vi "Test Comm CAN.vi"() -> ()   [LabVIEW 2021]
uses:
  <vilib>/CIF Foundation/CIF Channels Core/ChannelCommon/typedef/Direction.ctl
  CIF_CIPC_CAN.lvclass
  <vilib>/CIF Foundation/CIF Channels Core/ChannelCommon/typedef/FIFO Config.ctl
  <vilib>/CIF Foundation/CIF Channels Core/ChannelCommon/typedef/TimeStamps.ctl
  <vilib>/CIF Foundation/CIF Channels Core/ChannelCommon/typedef/New FIFO Instance Configuration.ctl
  <vilib>/CIF Foundation/CIF Channels Core/ChannelCommon/ChannelCommon.lvlib
panel:
  out "status":string
  out "pass":bool
  out "error out":errorcluster
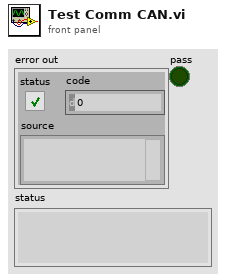
[diagram p1: front panel]
types:
  T1 = typedef "ChannelCommon.lvlib/Direction.ctl" = enum8{"Publisher", "Subscriber"}
  T2 = typedef "ChannelCommon.lvlib/New FIFO Instance Configuration.ctl" = cluster{"Backpressure":bool, "Bytes/Message Override":u32, "Messages/FIFO Override":u32, "Custom Data":u8[]}
  T3 = typedef "ChannelCommon.lvlib/TimeStamps.ctl" = cluster{"ClockID":u8, "T0":i64, "T_Out":i64}
  T4 = typedef "ChannelCommon.lvlib/FIFO Config.ctl" = cluster{"Max Bytes/Msg":u64, "Max Msg/FIFO":u64, "Flags":u64, "Custom Data":u8[]}
  T5 = typedef "ChannelCommon.lvlib/New FIFO Instance Response.ctl" = cluster{"Publisher":string, "Custom Data":u8[]}
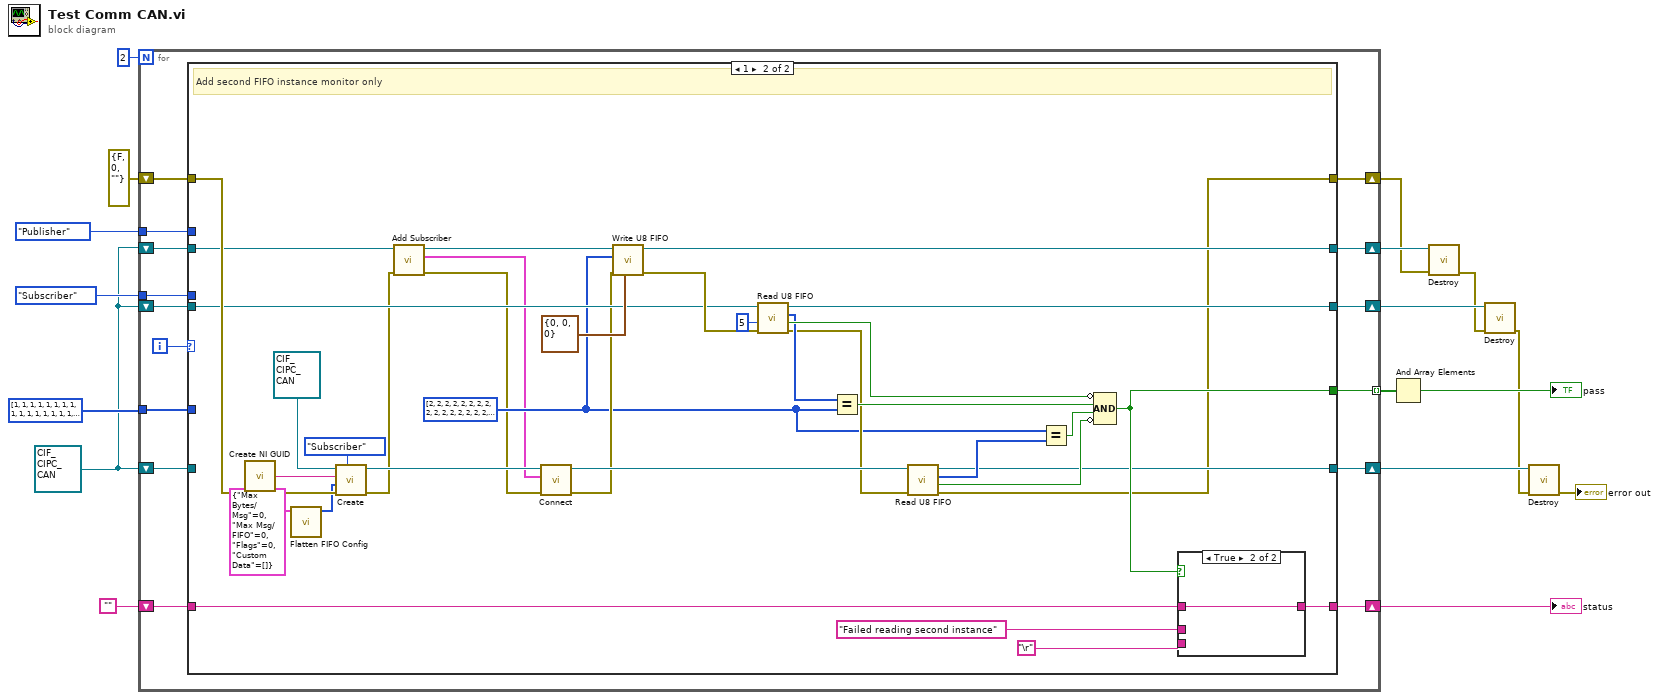
[diagram p0: block diagram]
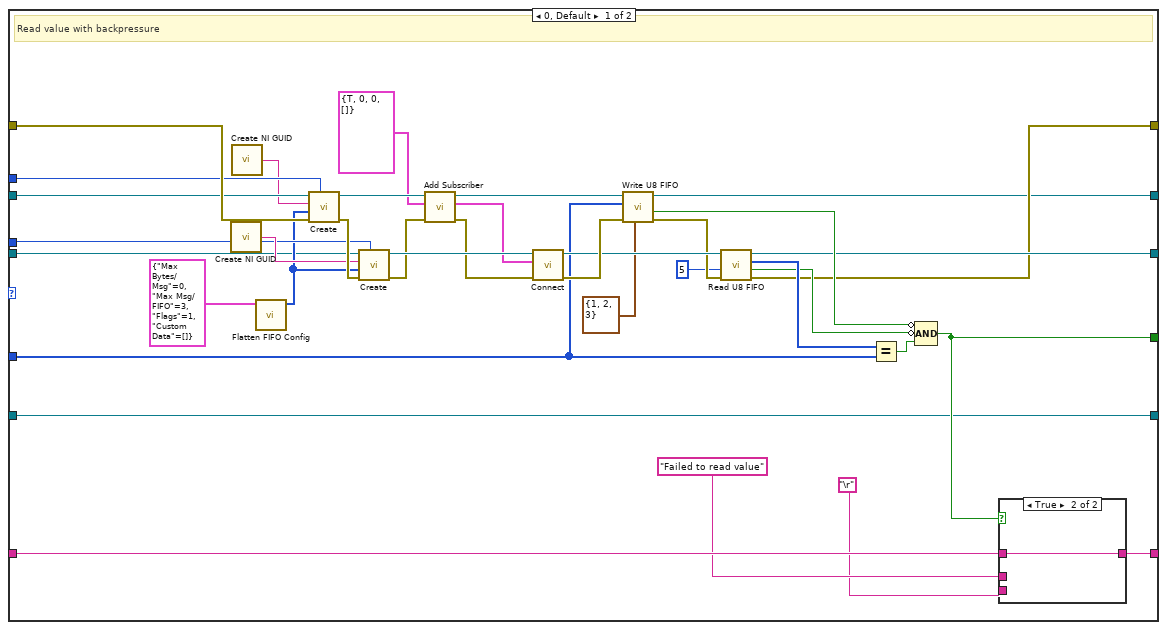
[diagram p2: hidden frame]
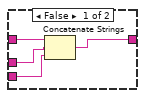
[diagram p3: hidden frame]
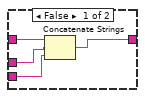
[diagram p4: hidden frame]
diagram:
  w1 = refnum<class "CIF_CIPC_CAN.lvclass"> refnum ("CIF_DAQ_DVR_Multi.lvclass")
  n1 = for {
    N: 2 -> [_]
    tunnel: [w32] -> w17 mode=indexing
    shift-right: [w25] -> w7
    shift-left: errorcluster {"status"=FALSE, "code"=0, "source"=""} ("error out") -> [w31]
    shift-right: [w28] -> w13
    shift-left: "" -> [w29]
    tunnel: Direction."Subscriber" ("Direction") -> [w27]
    tunnel: Direction."Publisher" ("Direction") -> [w26]
    shift-right: [w20] -> w9
    shift-left: w1 -> [w24]
    shift-right: [w19] -> w8
    shift-left: w1 -> [w18]
    tunnel: u8[] [1, 1, 1, 1, 1, 1, 1, 1, 1, 1, 1, 1, 1, 1, 1, 1, 1, 1, 1, 1, 1, 1, 1, 1, 1, 1, 1, 1, 1, 1, 1, 1, 1, 1, 1, 1, 1, 1, 1, 1, 1, 1, 1, 1, 1, 1, 1, 1, 1, 1, 1] ("Data in") -> [w23]
    shift-right: [w21] -> w5
    shift-left: w1 -> [w22]
    i -> [w30]
    n2 = case shown="1" w30 {
      tunnel: [w63 w104] -> w32
      tunnel: w31 -> [w61 w94]
      tunnel: [w42 w80] -> w25
      tunnel: w29 -> [w68 w108]
      tunnel: [w67 w107] -> w28
      tunnel: w27 -> [w59 _]
      tunnel: w26 -> [w58 _]
      tunnel: [w43 w86] -> w20
      tunnel: [w40 w84] -> w19
      tunnel: w18 -> [w48 w78]
      tunnel: w24 -> [w47 w85]
      tunnel: w23 -> [w41 _]
      tunnel: w22 -> [w46 _]
      tunnel: [w46 w87] -> w21
      frame 0, Default {
        # "Read value with backpressure"
        n3 = call <vilib>:"Create NI GUID.vi"() -> ("NI GUID"=w60:string)
        n4 = call <vilib>:"Create NI GUID.vi"() -> ("NI GUID"=w37:string)
        n5 = call <vilib>:"Flatten FIFO Config.vi"("FIFO Config in"=T4 {"Max Bytes/Msg"=0, "Max Msg/FIFO"=3, "Flags"=1, "Custom Data"=[]}) -> ("Flattened FIFO Config"=w55:u8[])  [unwired: 10 in]
        n6 = call-dynamic "Create.vi"("Direction"=w58, "error in (no error)"=w61, "Custom Config Data"=w55, "Name"=w37, "CIFFIFO in"=w48) -> ("error out"=w62:errorcluster, "CIFFIFO out"=w39:refnum<class "CIF_CIPC_CAN.lvclass">)  [unwired: 5 in]
        n7 = call-dynamic "Create.vi"("Direction"=w59, "error in (no error)"=w62, "Custom Config Data"=w55, "Name"=w60, "CIFFIFO in"=w47) -> ("error out"=w34:errorcluster, "CIFFIFO out"=w56:refnum<class "CIF_CIPC_CAN.lvclass">)  [unwired: 5 in]
        n8 = call-dynamic "Add Subscriber.vi"("error in (no error)"=w34, "New FIFO Instance Config"=T2 {"Backpressure"=TRUE, "Bytes/Message Override"=0, "Messages/FIFO Override"=0, "Custom Data"=[]}, "CIF_CIPC_Chn in"=w39) -> ("error out"=w33:errorcluster, "New FIFO Instance"=w36:T5, "CIF_CIPC_Chn out"=w38:refnum<class "CIF_CIPC_CAN.lvclass">)  [unwired: 6 in]
        n9 = call-dynamic "Connect.vi"("error in (no error)"=w33, "Connection"=w36, "CIFTag in"=w56) -> ("error out"=w54:errorcluster, "CIFTag out"=w52:refnum<class "CIF_CIPC_CAN.lvclass">)  [unwired: 7 in]
        n10 = call-dynamic "Write U8 FIFO.vi"("FIFO Timestamps"=T3 {"ClockID"=1, "T0"=2, "T_Out"=3}, "error in (no error)"=w54, "Data in"=w41, "CIFFIFO in"=w38) -> ("error out"=w49:errorcluster, "timed out?"=w53:bool, "CIFFIFO out"=w40:refnum<class "CIF_CIPC_CAN.lvclass">)  [unwired: 4 in, 1 out]
        n11 = call-dynamic "Read U8 FIFO.vi"("error in (no error)"=w49, "Timeout (ms)"=5, "CIFFIFO in"=w52) -> ("error out"=w42:errorcluster, "timed out?"=w50:bool, "Data out"=w51:u8[], "CIFFIFO out"=w43:refnum<class "CIF_CIPC_CAN.lvclass">)  [unwired: 4 in, 1 out]
        n12 = Equal?(x=w51, y=w41) -> (x = y?=w64:bool)
        n13 = Compound Arithmetic op=AND(invert w53, invert w50, w64) -> (w63:bool)
        n14 = case shown="True" w63 {
          tunnel: w68 -> [w72 w73]
          tunnel: [w69 w73] -> w67
          tunnel: "Failed to read value" -> [w71 _]
          tunnel: "\r" -> [w70 _]
          frame False {
            n15 = Concatenate Strings(w72, w71, w70) -> (w69:string)
          }
          frame True {
          }
        }
      }
      frame 1 {
        w79 = u8[] [2, 2, 2, 2, 2, 2, 2, 2, 2, 2, 2, 2, 2, 2, 2, 2, 2, 2, 2, 2, 2, 2, 2, 2, 2, 2, 2, 2, 2, 2, 2, 2, 2, 2, 2, 2, 2, 2, 2, 2, 2, 2, 2, 2, 2, 2, 2, 2, 2, 2, 2] ("Data in")
        # "Add second FIFO instance monitor only"
        n16 = call <vilib>:"Create NI GUID.vi"() -> ("NI GUID"=w96:string)
        n17 = call <vilib>:"Flatten FIFO Config.vi"("FIFO Config in"=T4 {"Max Bytes/Msg"=0, "Max Msg/FIFO"=0, "Flags"=0, "Custom Data"=[]}) -> ("Flattened FIFO Config"=w93:u8[])  [unwired: 10 in]
        n18 = call-dynamic "Create.vi"("Direction"=Direction."Subscriber", "error in (no error)"=w94, "Custom Config Data"=w93, "Name"=w96, "CIFFIFO in"=refnum<class "CIF_CIPC_CAN.lvclass"> refnum ("CIF_DAQ_DVR_Multi.lvclass")) -> ("error out"=w77:errorcluster, "CIFFIFO out"=w95:refnum<class "CIF_CIPC_CAN.lvclass">)  [unwired: 5 in]
        n19 = call-dynamic "Add Subscriber.vi"("error in (no error)"=w77, "CIF_CIPC_Chn in"=w78) -> ("error out"=w76:errorcluster, "New FIFO Instance"=w75:T5, "CIF_CIPC_Chn out"=w74:refnum<class "CIF_CIPC_CAN.lvclass">)  [unwired: 7 in]
        n20 = call-dynamic "Connect.vi"("error in (no error)"=w76, "Connection"=w75, "CIFTag in"=w95) -> ("error out"=w82:errorcluster, "CIFTag out"=w83:refnum<class "CIF_CIPC_CAN.lvclass">)  [unwired: 7 in]
        n21 = call-dynamic "Write U8 FIFO.vi"("FIFO Timestamps"=T3 {"ClockID"=0, "T0"=0, "T_Out"=0}, "error in (no error)"=w82, "Data in"=w79, "CIFFIFO in"=w74) -> ("error out"=w89:errorcluster, "CIFFIFO out"=w84:refnum<class "CIF_CIPC_CAN.lvclass">)  [unwired: 4 in, 2 out]
        n22 = call-dynamic "Read U8 FIFO.vi"("error in (no error)"=w89, "Timeout (ms)"=5, "CIFFIFO in"=w85) -> ("error out"=w81:errorcluster, "timed out?"=w100:bool, "Data out"=w99:u8[], "CIFFIFO out"=w86:refnum<class "CIF_CIPC_CAN.lvclass">)  [unwired: 4 in, 1 out]
        n23 = Equal?(x=w99, y=w79) -> (x = y?=w102:bool)
        n24 = call-dynamic "Read U8 FIFO.vi"("error in (no error)"=w81, "CIFFIFO in"=w83) -> ("error out"=w80:errorcluster, "timed out?"=w88:bool, "Data out"=w90:u8[], "CIFFIFO out"=w87:refnum<class "CIF_CIPC_CAN.lvclass">)  [unwired: 5 in, 1 out]
        n25 = Equal?(x=w79, y=w90) -> (x = y?=w103:bool)
        n26 = Compound Arithmetic op=AND(invert w100, w102, w103, invert w88) -> (w104:bool)
        n27 = case shown="True" w104 {
          tunnel: w108 -> [w112 w113]
          tunnel: [w109 w113] -> w107
          tunnel: "Failed reading second instance" -> [w111 _]
          tunnel: "\r" -> [w110 _]
          frame False {
            n28 = Concatenate Strings(w112, w111, w110) -> (w109:string)
          }
          frame True {
          }
        }
      }
    }
  }
  "status" <- w13
  n29 = And Array Elements(Boolean array=w17) -> (logical AND=→"pass":bool)
  n30 = call-dynamic "Destroy.vi"("error in (no error)"=w7, "CIFTag in"=w8) -> ("error out"=w6:errorcluster)  [unwired: 8 in, 1 out]
  n31 = call-dynamic "Destroy.vi"("error in (no error)"=w6, "CIFTag in"=w9) -> ("error out"=w4:errorcluster)  [unwired: 8 in, 1 out]
  n32 = call-dynamic "Destroy.vi"("error in (no error)"=w4, "CIFTag in"=w5) -> ("error out"=→"error out":errorcluster)  [unwired: 8 in, 1 out]
